vi "Migrate Dependencies.vi"(0 "project path":path, 5 "measurement paths":path[](array[path]), 7 "plug-in names":string[](array[string]), 9 "progress":refnum<vi>, 11 "error in":errorcluster) -> (4 "instrument containing sub vis":path[][](array[path]), 15 "error out":errorcluster)   [LabVIEW 2021, in "Multiple Converter.lvlib"]
doc: "Convert multiple measurements along with their dependencies, either dependencies being shared among measurements or measurements having their own depenencies."
uses:
  Multiple Converter.lvlib
panel:
  # "Dependencies Migration"
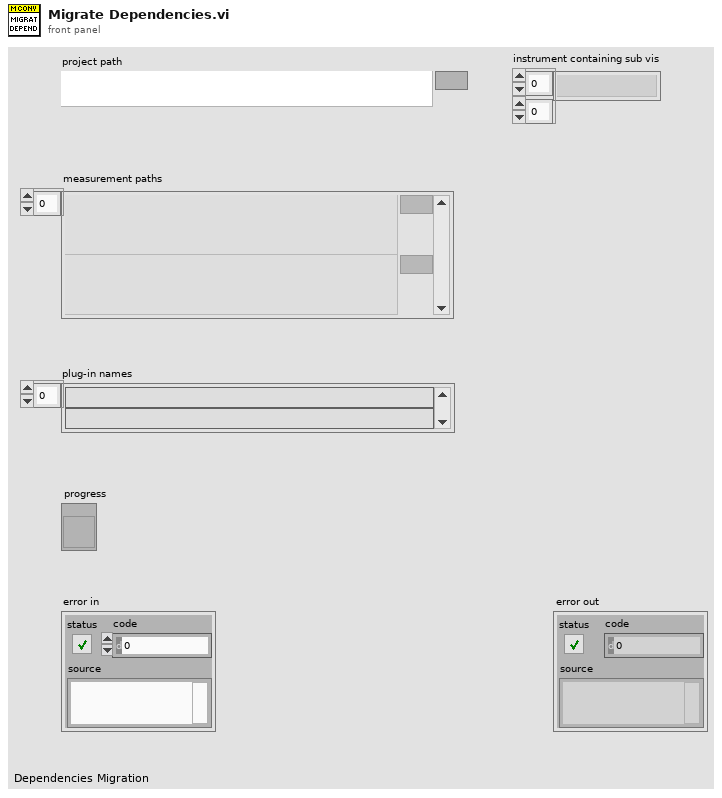
[diagram p1: front panel]
types:
  T1 = typedef "Multiple Converter.lvlib/Library Info.ctl" = cluster{"library path":path, "library name":string}
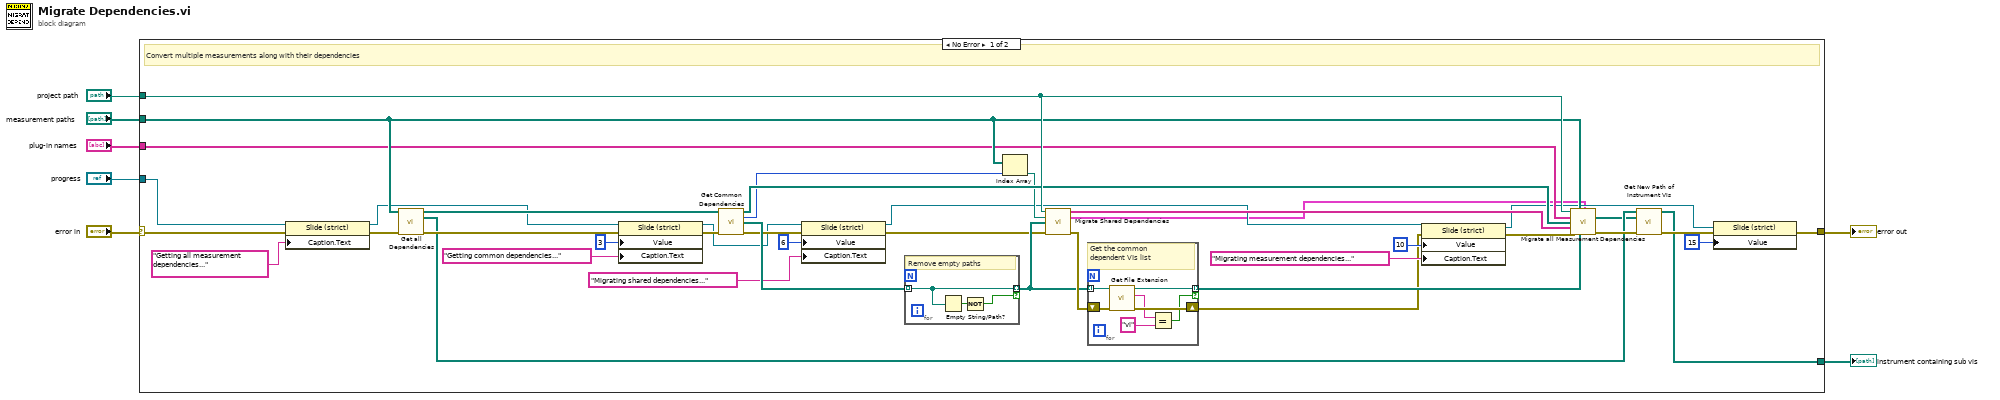
[diagram p0: block diagram]
diagram:
  n1 = case shown="No Error" "error in" {
    selector: "error in" -> [w35 w58]
    tunnel: "project path" -> [w47 _]
    tunnel: "measurement paths" -> [w46 _]
    tunnel: "plug-in names" -> [w45 _]
    tunnel: [w17 w58] -> w4
    tunnel: [w11 _] -> w2
    tunnel: "progress" -> [w33 _]
    frame No Error {
      # "Convert multiple measurements along with their dependencies"
      n2 = property class="Slide (strict)"(reference=w33, error in=w35, "Caption.Text"="Getting all measurement dependencies...") -> (reference out=w29:refnum<vi>, error out=w34:errorcluster)
      n3 = call "Get all Dependencies.vi"("measurement paths"=w46, "error in"=w34) -> ("all dependencies"=w44:path[][], "instrument containing sub vis"=w12:path[][], "error out"=w32:errorcluster)  [unwired: 11 in]
      n4 = property class="Slide (strict)"(reference=w29, error in=w32, "Value"=3, "Caption.Text"="Getting common dependencies...") -> (reference out=w23:refnum<vi>, error out=w31:errorcluster)
      n5 = call "Get Common Dependencies.vi"("all dependencies"=w44, "error in"=w31) -> ("measurement dependencies"=w43:path[][], "measurement index"=w37:i32, "common dependencies"=w38:path[], "error out"=w25:errorcluster)  [unwired: 10 in]
      n6 = property class="Slide (strict)"(reference=w23, error in=w25, "Value"=6, "Caption.Text"="Migrating shared dependencies...") -> (reference out=w16:refnum<vi>, error out=w24:errorcluster)
      n7 = for {
        tunnel: [w48] -> w36 mode=indexing if=w49
        tunnel: w38 -> [w48] mode=indexing
        # "Remove empty paths"
        n8 = Empty String/Path?(string/path=w48) -> (empty?=w50:bool)
        n9 = Not(x=w50) -> (.not. x?=w49:bool)
      }
      n10 = Index Array(array=w46, index=w37) -> (element=w39:path)
      n11 = call "Migrate Shared Dependencies.vi"("project path"=w47, "measurement path"=w39, "common dependencies"=w36, "error in"=w24) -> ("outside items"=w42:string[], "library"=w9:T1[], "error out"=w40:errorcluster)  [unwired: 9 in]
      n12 = for {
        shift-right: [w56] -> w20
        shift-left: w40 -> [w57]
        tunnel: [w52] -> w41 mode=indexing if=w53
        tunnel: w36 -> [w51] mode=indexing
        # "Get the common dependent VIs list"
        n13 = call <vilib>:"Get File Extension.vi"("error in (no error)"=w57, "file"=w51) -> ("error out"=w56:errorcluster, "lowercase file extension"=w54:string, "dup file"=w52:path)  [unwired: 5 in, 2 out]
        n14 = Equal?(x=w54, y="vi" ("x")) -> (x = y?=w53:bool)
      }
      n15 = property class="Slide (strict)"(reference=w16, error in=w20, "Value"=10, "Caption.Text"="Migrating measurement dependencies...") -> (reference out=w15:refnum<vi>, error out=w19:errorcluster)
      n16 = call "Migrate all Measurement Dependencies.vi"("project path"=w47, "measurement paths"=w46, "init"=w9, "plug-in names"=w45, "measurement dependencies"=w43, "outside items"=w42, "error in"=w19, "shared dependent vis"=w41) -> ("destination directory"=w10:path[], "error out"=w14:errorcluster)  [unwired: 6 in]
      n17 = call "Get New Path of Instrument VIs.vi"("instr containing vis"=w12, "destination directory"=w10, "error in"=w14) -> ("new path of instr containing vis"=w11:path[][], "error out"=w13:errorcluster)  [unwired: 11 in]
      n18 = property class="Slide (strict)"(reference=w15, error in=w13, "Value"=15) -> (error out=w17:errorcluster)  [unwired: 1 out]
    }
    frame Error {
    }
  }
  "error out" <- w4
  "instrument containing sub vis" <- w2
